vi "SubSystems.vi"(8 "error in":errorcluster) -> ()   [LabVIEW 2017]
doc: "This VI calls the various robot subsystems that will then run in parallel. New subSystems will automatlically script code to make the call."
uses:
  <vilib>/Rock Robotics/SystemInterfaces/DIO/FPGA_DIOPWMChannel.ctl
  <vilib>/Rock Robotics/WPI/DriverStation/WPI_DriverStationRobotMode2.ctl
  <vilib>/Rock Robotics/WPI/RobotDrive/WPI_RobotDriveOpen2MotorWithSPARK.vi
  Framework/Robot Global Data.vi
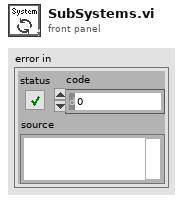
[diagram p1: front panel]
types:
  T1 = typedef "FPGA_DIOPWMChannel.ctl" = enum8{"PWM 0", "PWM 1", "PWM 2", "PWM 3", "PWM 4", "PWM 5", "PWM 6", "PWM 7", "PWM 8", "PWM 9", "PWM MXP 0", "PWM MXP 1", "PWM MXP 2", "PWM MXP 3", "PWM MXP 4", "PWM MXP 5", "PWM MXP 6", "PWM MXP 7", "PWM MXP 8", "PWM MXP 9", "Invalid"}
  T2 = typedef "WPI_RobotDriveDevRef.ctl" = cluster{"DevStatus":errorcluster, "Motors[]":T3[], "Square Inputs":bool, "Max Output":dbl}
  T3 = typedef "WPI_MotorControlDeviceRef.ctl" = cluster{"DeviceStatus":errorcluster, "Type":T4, "PWM":cluster{"PWM Channel":T1, "DeadBand":T5}, "CAN":cluster{"Device Number":u8, "SetOutput VI Ref":variant, "GetOutput VI Ref":variant, "Enable VI Ref":variant, "Disable VI Ref":variant, "Data":variant}, "Invert":bool, "DIO PWM":cluster{"PWM \"Enable\" Channel":T1, "DIOChannel":T6, "PWM Rate":dbl}}
  T4 = typedef "WPI_MotorControlType.ctl" = enum16{"PWM", "CAN", "DIO PWM"}
  T5 = typedef "WPI_PWMDeadband.ctl" = cluster{"Name":string, "maxPositivePwm":i32, "minPositivePwm":i32, "centerPwm":i32, "maxNegativePwm":i32, "minNegativePwm":i32, "angularRange":u16}
  T6 = typedef "FPGA_DIOChannel.ctl" = enum8{"DIO 0", "DIO 1", "DIO 2", "DIO 3", "DIO 4", "DIO 5", "DIO 6", "DIO 7", "DIO 8", "DIO 9", "DIO MXP 0", "DIO MXP 1", "DIO MXP 2", "DIO MXP 3", "DIO MXP 4", "DIO MXP 5", "DIO MXP 6", "DIO MXP 7", "DIO MXP 8", "DIO MXP 9", "DIO MXP 10", "DIO MXP 11", "DIO MXP 12", "DIO MXP 13", "DIO MXP 14", "DIO MXP 15", "SPI Port CS1", "SPI Port CS2", "SPI Port CS3", "SPI Port MISO", "SPI Port MOSI", "Invalid"}
  T7 = typedef "WPI_DriverStationRobotMode2.ctl" = enum16{"Autonomous Disabled", "Autonomous Enabled", "Teleop Disabled", "Teleop Enabled", "Disconnected", "Finish", "Test Disabled", "Test Enabled", "Emergency Stopped"}
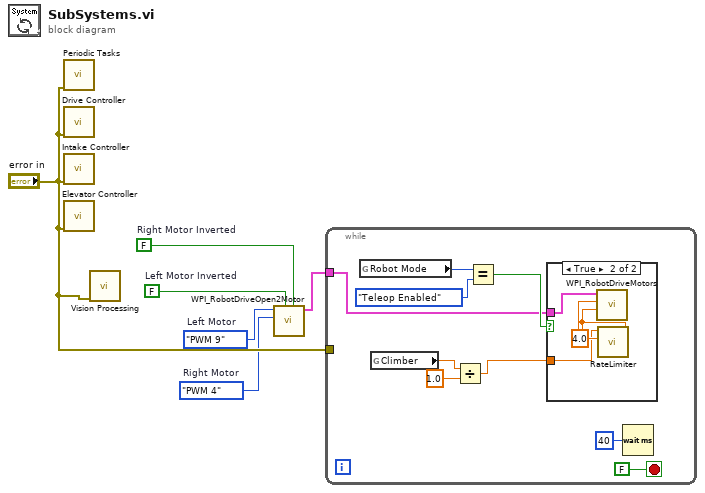
[diagram p0: block diagram]
diagram:
  w1 = FPGA_DIOPWMChannel."PWM 9"  # Left Motor
  w2 = FPGA_DIOPWMChannel."PWM 4"  # Right Motor
  w3 = FALSE  # Left Motor Inverted
  w4 = FALSE  # Right Motor Inverted
  n1 = call "Periodic Tasks.vi"("error in"="error in") -> ()  [unwired: 1 in, 10 out]
  n2 = call "Drive Controller.vi"("error in"="error in") -> ()  [unwired: 11 in]
  n3 = call "Intake Controller.vi"("error in"="error in") -> ()  [unwired: 11 in]
  n4 = call "Elevator Controller.vi"("error in"="error in") -> ()  [unwired: 11 in]
  n5 = call "Vision Processing.vi"("error in (no error)"="error in") -> ()  [unwired: 7 in]
  n6 = call-poly <vilib>:"WPI_RobotDriveOpen2Motor.vi"("Right Motor Inverted"=w4, "Left Motor Inverted"=w3, "Right Motor"=w2, "Left Motor"=w1) -> ("RobotDriveDevRef"=w5:T2)  [unwired: 6 in, 1 out]
  n7 = while {
    tunnel: "error in" -> [_]
    tunnel: w5 -> [w10]
    stop <- FALSE stop-if-true
    n8 = global read "Robot Global Data.vi" "Robot Mode"() -> (w13:T7)
    n9 = global read "Robot Global Data.vi" "Climber"() -> (w9:dbl)
    n10 = Divide(x=w9, y=1.0) -> (x/y=w7:dbl)
    n11 = Equal?(x=w13, y=WPI_DriverStationRobotMode2."Teleop Enabled") -> (x = y?=w11:bool)
    n12 = case shown="True" w11 {
      tunnel: w10 -> [_ w19]
      tunnel: w7 -> [_ w16]
      frame False {
      }
      frame True {
        n13 = call "RateLimiter.vi"("Max dx/dt"=4.0, "Input"=w16) -> ("Output"=w18:dbl)  [unwired: 9 in]
        n14 = call <vilib>:"WPI_RobotDriveMotors.vi"("RightSpeed"=w18, "LeftSpeed"=w18, "RobotDriveDevRef"=w19) -> ()  [unwired: 6 in, 3 out]
      }
    }
    n15 = Wait (ms)(milliseconds to wait=u32 40) -> ()  [unwired: 1 out]
  }
